vi "Table_AllItems_Tests.vi"(8 "error in":errorcluster) -> (0 "error out":errorcluster)   [LabVIEW 2016, in "DronaTest.lvlib"]
uses:
  DronaTest.lvlib
  APIs/Stimulus/ControlValue/SetValueAuto.vi
  APIs/Stimulus/ControlValue/Controls/Table/SetValue.vi
  APIs/Assert/AssertControlValue/Controls/Table/AssertAllItems.vi
  <vilib>/addons/_JKI Toolkits/Caraya/classes/Assert/Assert Error.vi
  <vilib>/addons/_JKI Toolkits/Caraya/classes/Test/Test.lvclass
  <vilib>/SLL Toolkit/SLL Debug/SLL Debug.lvlib
  Drona.lvlib
  <vilib>/addons/_JKI Toolkits/Caraya/classes/Assert/Assert.lvclass
  APIs/Stimulus/ControlValue/Controls/Table/StimulusTable.lvlib
  APIs/Stimulus/ControlValue/ControlValue.lvlib
  APIs/Assert/AssertControlValue/Controls/Table/AssertTable.lvlib
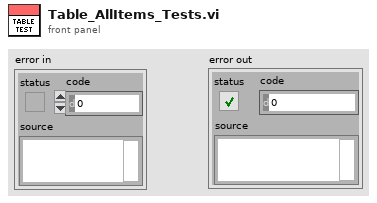
[diagram p1: front panel]
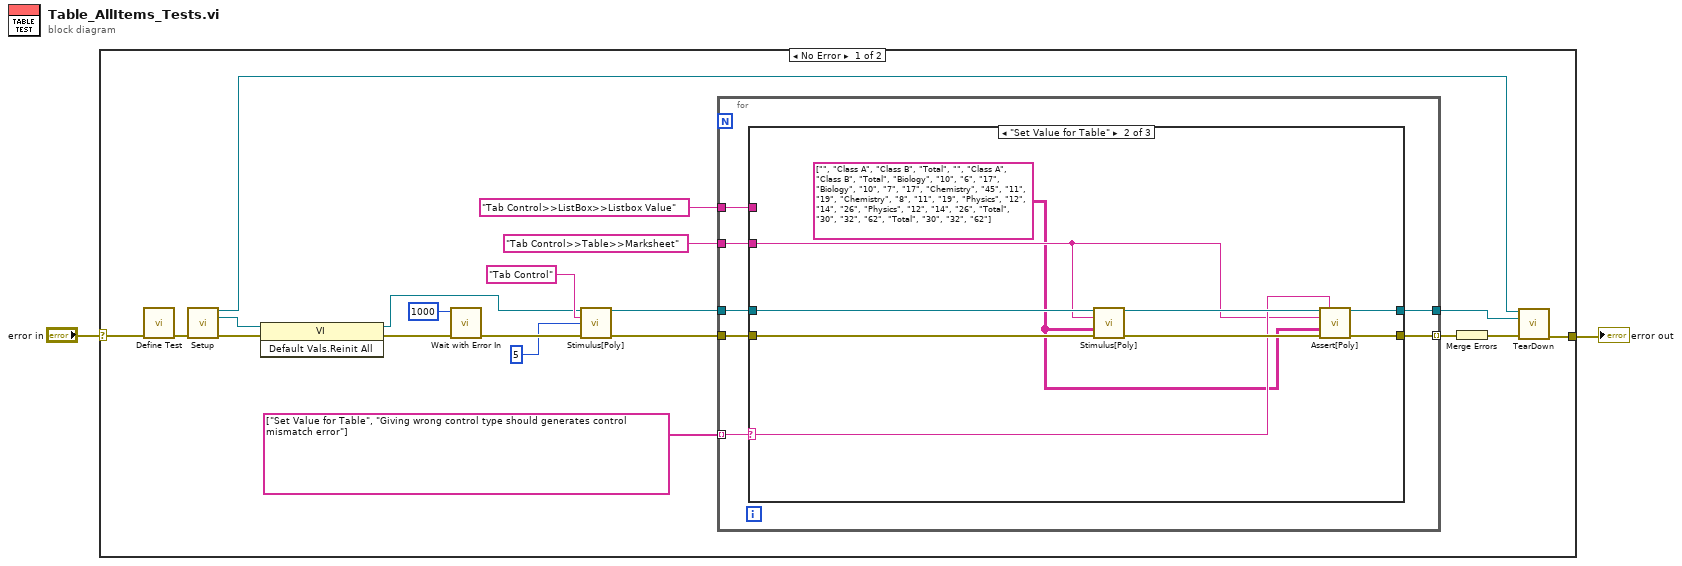
[diagram p0: block diagram]
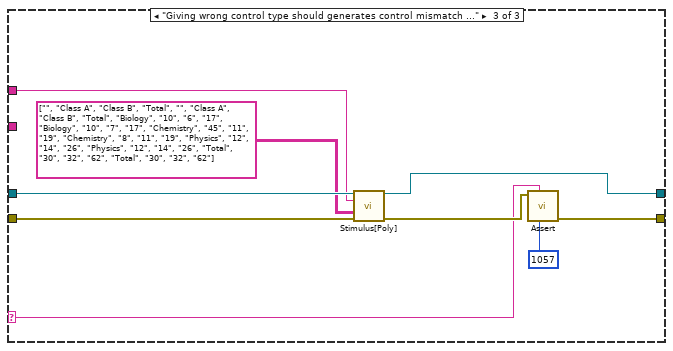
[diagram p3: hidden frame]
diagram:
  n1 = case shown="No Error" "error in" {
    selector: "error in" -> [w22 w50]
    tunnel: [w7 w50] -> w1
    frame No Error {
      n2 = call <vilib>:"Define Test.vi"("error in (no error)"=w22) -> ("error out"=w12:errorcluster)  [unwired: 9 in, 1 out]
      n3 = call "Setup.vi"("error in"=w12) -> ("Application Ref"=w9:refnum<vi>, "VI out"=w4:refnum<vi>, "error out"=w11:errorcluster)  [unwired: 12 in]
      n4 = invoke class="VI" method="Default Vals.Reinit All"(reference=w4, error in=w11) -> (reference out=w3:refnum<vi>, error out=w5:errorcluster)  [unwired: 1 in, 1 out]
      n5 = call <vilib>:"Wait with Error In.vi"("error in (no error)"=w5, "milliseconds to wait"=u32 1000) -> ("error out"=w20:errorcluster)  [unwired: 9 in]
      n6 = call-poly "Stimulus[Poly].vi"("VI Reference In"=w3, "Control Path"="Tab Control", "Value (Signaling)"=5, "error in"=w20) -> ("VI Reference Out"=w16:refnum<vi>, "error out"=w19:errorcluster)  [unwired: 10 in]
      n7 = for {
        tunnel: w16 -> [w28]
        tunnel: "Tab Control>>Table>>Marksheet" ("Control Path") -> [w27]
        tunnel: "Tab Control>>ListBox>>Listbox Value" ("Control Path") -> [w26]
        tunnel: string[] ["Set Value for Table", "Giving wrong control type should generates control mismatch error"] -> [w24] mode=indexing
        tunnel: [w23] -> w8
        tunnel: w19 -> [w29]
        tunnel: [w25] -> w13 mode=indexing
        n8 = case shown="\"Set Value for Table\"" w24 {
          selector: w24 -> [_ w34 w45]
          tunnel: w29 -> [w31 w40 w49]
          tunnel: w28 -> [w30 w39 w48]
          tunnel: w27 -> [_ w33 _]
          tunnel: w26 -> [_ _ w42]
          tunnel: [w31 w36 w46] -> w25
          tunnel: [w30 w35 w43] -> w23
          frame Default {
          }
          frame "Set Value for Table" {
            w32 = string[][] [["", "Class A", "Class B", "Total", "", "Class A", "Class B", "Total"], ["Biology", "10", "6", "17", "Biology", "10", "7", "17"], ["Chemistry", "45", "11", "19", "Chemistry", "8", "11", "19"], ["Physics", "12", "14", "26", "Physics", "12", "14", "26"], ["Total", "30", "32", "62", "Total", "30", "32", "62"]] ("Value")
            n9 = call-poly "Stimulus[Poly].vi"("VI Reference In"=w39, "Control Path"=w33, "Value"=w32, "Error In"=w40) -> ("VI Reference Out"=w37:refnum<vi>, "Error Out"=w38:errorcluster)  [unwired: 10 in]
            n10 = call-poly "Assert[Poly].vi"("VI Reference In"=w37, "Test Label"=w34, "Control Path"=w33, "Item Value"=w32, "Error In"=w38) -> ("VI Reference Out"=w35:refnum<vi>, "Error Out"=w36:errorcluster)  [unwired: 8 in, 1 out]
          }
          frame "Giving wrong control type should generates control mismatch error" {
            n11 = call-poly "Stimulus[Poly].vi"("VI Reference In"=w48, "Control Path"=w42, "Value"=string[][] [["", "Class A", "Class B", "Total", "", "Class A", "Class B", "Total"], ["Biology", "10", "6", "17", "Biology", "10", "7", "17"], ["Chemistry", "45", "11", "19", "Chemistry", "8", "11", "19"], ["Physics", "12", "14", "26", "Physics", "12", "14", "26"], ["Total", "30", "32", "62", "Total", "30", "32", "62"]], "Error In"=w49) -> ("VI Reference Out"=w43:refnum<vi>, "Error Out"=w47:errorcluster)  [unwired: 10 in]
            n12 = call-poly <vilib>:"Assert.vi"("error code (1)"=1057, "Label"=w45, "Error?"=w47) -> ("error out"=w46:errorcluster)  [unwired: 7 in, 1 out]
          }
        }
      }
      n13 = Merge Errors(w13) -> (w10:errorcluster)
      n14 = call "TearDown.vi"("Application Ref"=w9, "VI in"=w8, "error in (no error)"=w10) -> ("error out"=w7:errorcluster)  [unwired: 12 in]
    }
    frame Error {
    }
  }
  "error out" <- w1
